vi "RemoteVI Complex Fixture Button Refs.vi"(0 "Controls":refnum<vi>[](array[refnum])) -> (4 "Stop Ref":refnum<vi>, 5 "Inspector Ref":refnum<vi>, 6 "View Ref":refnum<vi>, 7 "Data File Ref":refnum<vi>)   [LabVIEW 2020]
doc: "Helper of RemoteVI Complex Fixture Events.vi. Splits the array of control references RemoteVI Complex Fixture Find Controls.vi returns for Stop, Inspector, View, Data File into one named reference each, so Register For Events names each event source after its control (<Stop Ref>)."
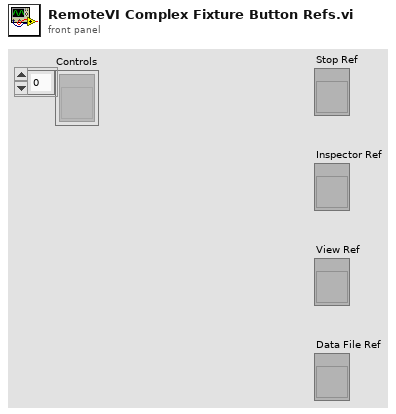
[diagram p1: front panel]
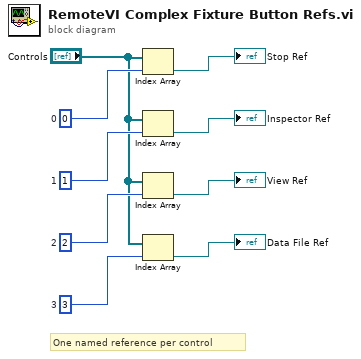
[diagram p0: block diagram]
diagram:
  w8 = 3  # 3
  w6 = 2  # 2
  w4 = 1  # 1
  w2 = 0  # 0
  # "One named reference per control"
  n1 = Index Array(array="Controls", index=w2) -> (element=→"Stop Ref":refnum<vi>)
  n2 = Index Array(array="Controls", index=w4) -> (element=→"Inspector Ref":refnum<vi>)
  n3 = Index Array(array="Controls", index=w6) -> (element=→"View Ref":refnum<vi>)
  n4 = Index Array(array="Controls", index=w8) -> (element=→"Data File Ref":refnum<vi>)
